vi "PicoScope5000aExampleRapidBlockBulkOverlapped.vi"() -> ()   [LabVIEW 2010]
uses:
  shared/PicoBuffers.ctl
  <vilib>/Waveform/DWDTOps.llb/DWDT Analog to Digital.vi
  PicoScope5000aLib/PicoScope5000aAnalogChannelSettings.ctl
  shared/Segment Range.ctl
  shared/Buffer and Transfer Settings.ctl
  shared/Acquisition Settings.ctl
  shared/nSegments.ctl
  PicoScope5000aLib/PicoScope5000aDigitalChannelSettings.ctl
panel:
  in  "Write TDMS file":bool
  out "Total Requested Samples":u64
  out "overflow":i16[](array[numeric]) format="%06b"
  in  "Port 0 Settings":T1={"Enabled"=FALSE, "Logic Level"=9830} {"Logic Level" items=["1.5V TTL"=9830, "2.5V CMOS"=16383]}
  in  "Channel A Settings":T2={"Enabled"=TRUE, "Coupling"=1, "Range"=6, "Analogue Offset"=0.0, "Bandwidth Limit"=0} {"Bandwidth Limit" items=["Full", "20MHz"]; "Range" items=["10 mV", "20 mV", "50 mV", "100 mV", "200 mV", "500 mV", "1 V", "2 V", "5 V", "10 V", "20 V"]; "Coupling" items=["AC", "DC"]}
  in  "Trigger Settings":T3={"Trigger Enabled"=FALSE, "Trigger Source"=enum."Channel A", "Trigger Threshold (volts)"=0.0, "Trigger Direction"=2, "Trigger Delay (samples)"=0, "Auto Trigger Time (ms)"=1000} {"Trigger Direction" items=["Rising"=2, "Falling"=3]}
  out "USB 3.0 device on non-USB 3.0 Port":bool=TRUE
  out "USB Powered":bool=TRUE
  out "Device Info":T4={"Driver Version"="0", "USB Version"="0", "Hardware"="0", "Variant"="0", "Batch and Serial"="0", "Cal Date"="0", "Kernel Version"="0", "Digital HW Version"="0", "Analogue HW Version"="0", "MSO"=FALSE, "Number of channels"=0}
  out "Trigger Offsets":cluster{"Samples":u64, "Time (seconds)":sgl}[](array[cluster]) {"Time (seconds)" format="%#_5p"}
  in  "Stop Display":bool
  out "Capture Complete":bool
  in  "Run":bool
  in  "Display Buffer Index":i32
  in  "Segment Range":T5={"fromSegmentIndex"=0, "toSegmentIndex"=9} {"toSegmentIndex" format="%.4p"; "fromSegmentIndex" format="%.4p"}
  in  "nSegments":T6=10 format="%.4p"
  out "error out":errorcluster
  in  "Data file":path=path "PicoScope5000aExampleRapidBlock"
  in  "Buffer and Transfer Settings":T7={"startIndex"=0, "Samples"=1000000, "Down Sample Ratio"=1, "Down-Sample Mode"=0} {"Down-Sample Mode" items=["None"=0, "Aggregate"=1, "Decimate"=2, "Average"=4, "RAW none"=2147483648]; "Down Sample Ratio" step=1; "Samples" format="%_6p"}
  in  "Acquisition Settings":T8={"preTriggerSamples"=0, "postTriggerSamples"=1000000, "timebase"=5} {"postTriggerSamples" format="%_6p"; "preTriggerSamples" format="%_6p"}
  out "Properties Panel":T9 {"Max Total Capture Time Available (sec)" format="%.3p"; "Sample Frequency" format="%.6p"; "Sample Rate" format="%.3p"; "Max Samples Available" format="%_6p"; "Total Capture Time (sec)" format="%.3p"}
  out "Port 0":digitalwaveform(graph)={"t0"=timestamp(0 s since 1904-01-01), "dt"=8e-09, "Y"={"transitions"=[], "data"=[]}}
  in  "stop":bool
  out "Analog Channels":cluster{i32, sgl, "Data":dbl[]}[](graph)
  in  "Resolution":u32(ring) items=["8-bit"=0, "12-bit"=1, "14-bit"=2, "15-bit"=3, "16-bit"=4, "10-bit"=10]
  in  "Serial Number":string
  in  "Use Serial Number":bool
  in  "error in (no error)":errorcluster
  # "Number of\nSegments to Capture"
  # "Bit 0 = ChA"
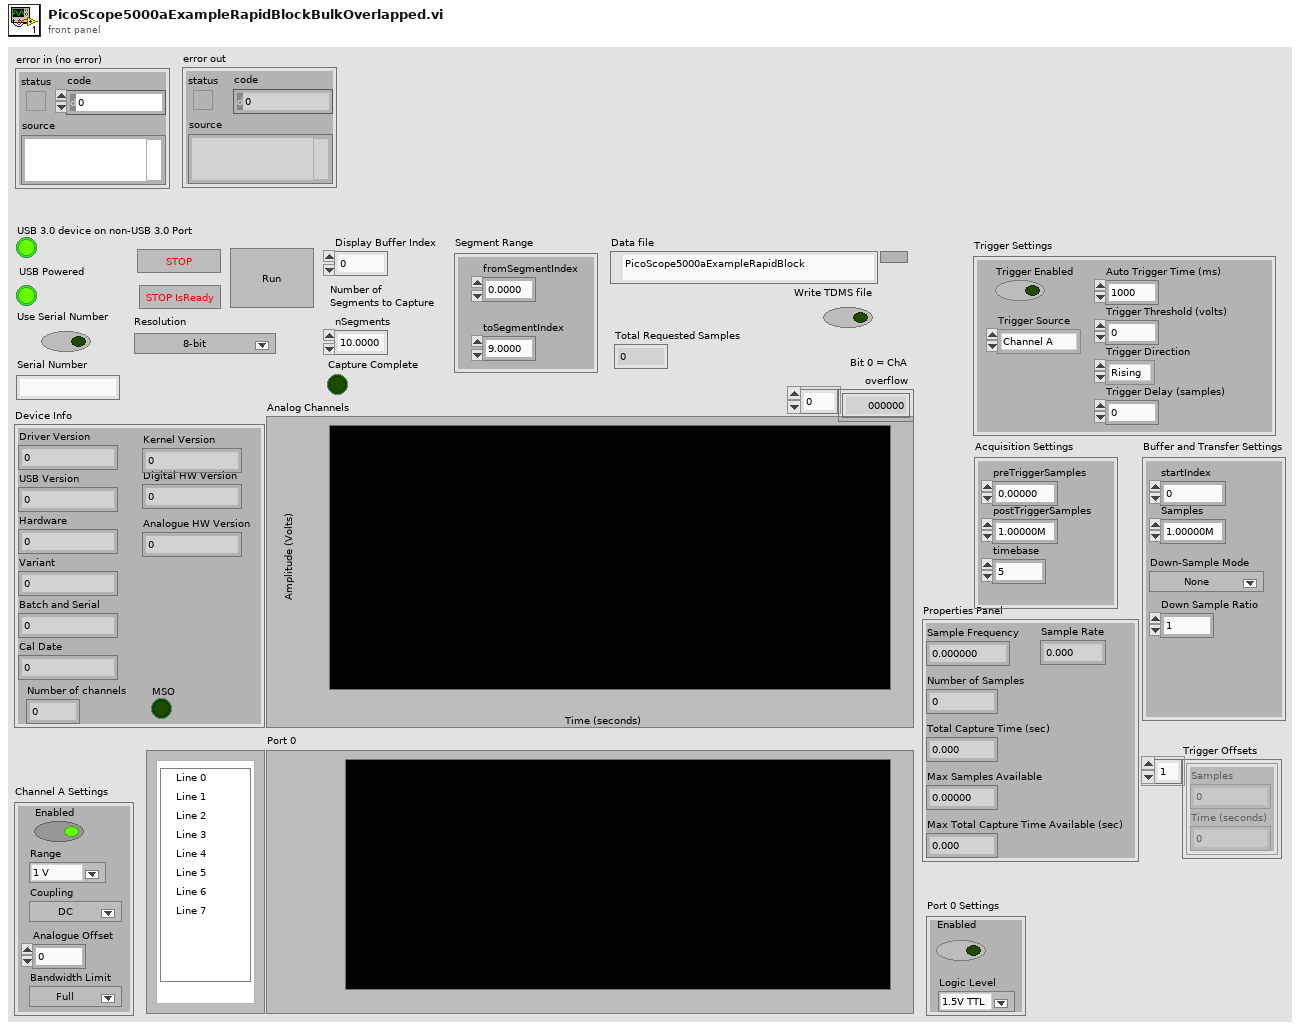
[diagram p1: front panel]
types:
  T1 = typedef "PicoScope5000aDigitalChannelSettings.ctl" = cluster{"Enabled":bool, "Logic Level":i16}
  T2 = typedef "PicoScope5000aAnalogChannelSettings.ctl" = cluster{"Enabled":bool, "Coupling":i16, "Range":u16, "Analogue Offset":sgl, "Bandwidth Limit":u32}
  T3 = cluster{"Trigger Enabled":bool, "Trigger Source":enum16{"Channel A", "Channel B", "Channel C", "Channel D", "Ext."}, "Trigger Threshold (volts)":dbl, "Trigger Direction":u16, "Trigger Delay (samples)":u32, "Auto Trigger Time (ms)":i16}
  T4 = cluster{"Driver Version":string, "USB Version":string, "Hardware":string, "Variant":string, "Batch and Serial":string, "Cal Date":string, "Kernel Version":string, "Digital HW Version":string, "Analogue HW Version":string, "MSO":bool, "Number of channels":i16}
  T5 = typedef "Segment Range.ctl" = cluster{"fromSegmentIndex":u64, "toSegmentIndex":u64}
  T6 = typedef "nSegments.ctl" = u64
  T7 = typedef "Buffer and Transfer Settings.ctl" = cluster{"startIndex":u64, "Samples":u64, "Down Sample Ratio":u64, "Down-Sample Mode":u32}
  T8 = typedef "Acquisition Settings.ctl" = cluster{"preTriggerSamples":u64, "postTriggerSamples":u64, "timebase":u32}
  T9 = cluster{"Sample Frequency":dbl, "Sample Rate":dbl, "Max Samples Available":u64, "Number of Samples":u64, "Total Capture Time (sec) ":dbl, "Max Total Capture Time Available (sec)":dbl}
  T10 = typedef "PicoBuffers.ctl" = cluster{"Max Buffer Pointers":u64[][][], "Min Buffer Pointers":u64[][][], "StreamingDataInfo":cluster{"Channel":u32, "Down-Sample Mode":u32, "PICO_DATA_TYPE":enum32{"PICO_INT8_T", "PICO_INT16_T", "PICO_INT32_T", "PICO_UINT32_T", "PICO_INT64_T", ""}, "Samples":i32, "bufferIndex":u64, "startIndex":i32, "overflow":i16}[][]}
  T11 = enum16{"open", "open or create", "create or replace", "create", "open (read-only)"}
  T12 = cluster{"Sample Frequency":sgl, "Sample Rate":sgl, "Max Samples Available":i32, "Number of Samples":u32, "Total Capture Time (sec) ":sgl, "Max Total Capture Time Available (sec)":sgl}
  T13 = cluster{"Channel A Buffer":i16[], "Channel B Buffer":i16[], "Channel C Buffer":i16[], "Channel D Buffer":i16[], "Channel E Buffer":i16[], "Channel F Buffer":i16[], "Channel G Buffer":i16[], "Channel H Buffer":i16[], "Port 0 Buffer":i16[], "Port 1 Buffer":i16[]}[]
  T14 = cluster{"Channel A Buffer":i16[], "Channel B Buffer":i16[], "Channel C Buffer":i16[], "Channel D Buffer":i16[], "Channel E Buffer":i16[], "Channel F Buffer":i16[], "Channel G Buffer":i16[], "Channel H Buffer":i16[], "Port 0 Buffer":i16[], "Port 1 Buffer":i16[]}
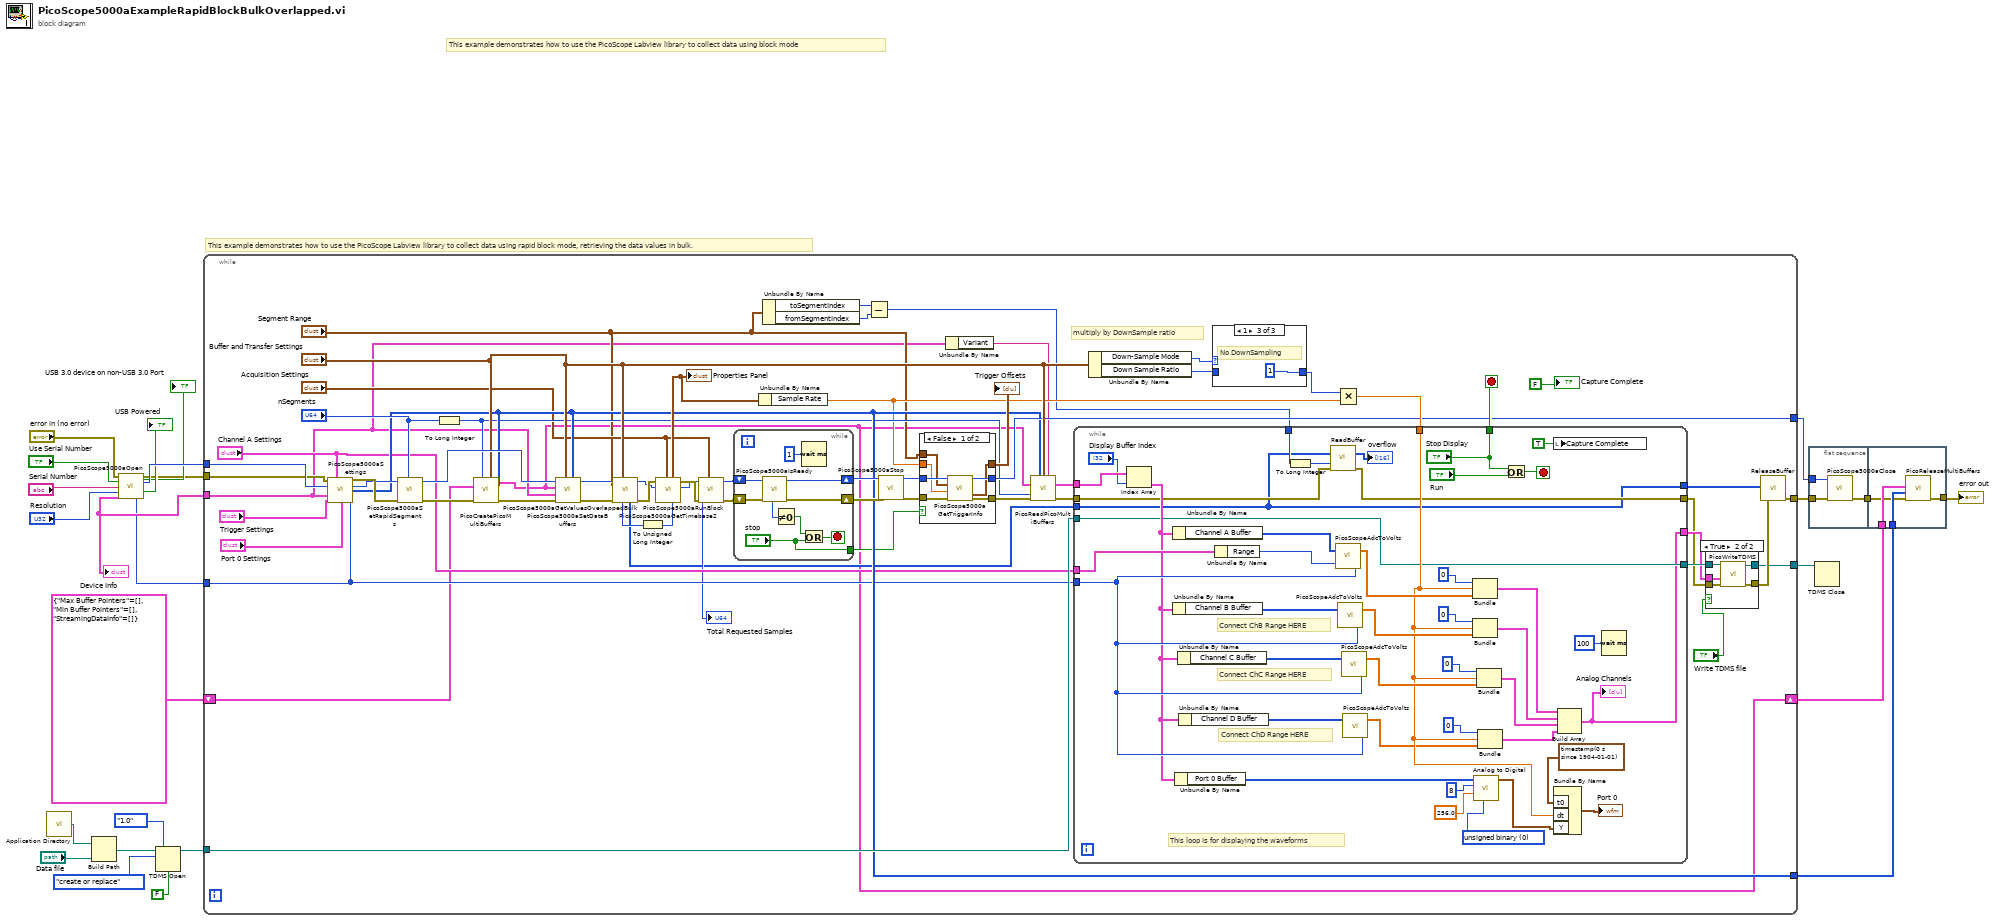
[diagram p0: block diagram]
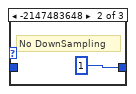
[diagram p5: hidden frame]
diagram:
  # "This example demonstrates how to use the PicoScope Labview library to collect data using rapid block mode, retrieving the data values in bulk."
  # "This example demonstrates how to use the PicoScope Labview library to collect data using block mode"
  n1 = call <vilib>:"Application Directory.vi"() -> ("Application Directory"=w19:path)
  n2 = Build Path(base path=w19, name or relative path="Data file") -> (appended path=w20:path)
  n3 = call "PicoScope5000aOpen.vi"("error in (no error)"="error in (no error)", "Serial Number"="Serial Number", "Use Serial Number"="Use Serial Number", "Resolution"="Resolution") -> ("USB 3.0 device on non-USB 3.0 Port"=→"USB 3.0 device on non-USB 3.0 Port":bool, "error out"=w8:errorcluster, "handle"=w25:i16, "USB Powered"=→"USB Powered":bool, "Device Info"=w12:T4, "Max ADC value"=w11:i16)  [unwired: 6 in]
  "Device Info" <- w12
  n4 = TDMS Open(6:FALSE ("disable buffering? (T)"), 7:enum16{"1.0", "2.0"}."1.0" ("file format version (2.0)"), 10:T11."create or replace" ("operation (0:open)"), 11:w20) -> (3:w17:refnum<k34>)  [unwired: 2 in, 1 out]
  n5 = while {
    tunnel: w25 -> [w56]
    tunnel: w11 -> [w48]
    tunnel: [w68] -> w6
    tunnel: [w53] -> w5
    tunnel: [w27] -> w18
    tunnel: w17 -> [w87]
    tunnel: w12 -> [w34]
    tunnel: w8 -> [w55]
    tunnel: [w41] -> w2
    shift-right: [w32] -> w4
    shift-left: T10 {"Max Buffer Pointers"=[], "Min Buffer Pointers"=[], "StreamingDataInfo"=[]} ("Data Pointers") -> [w33]
    stop <- w72 stop-if-true
    # "multiply by DownSample ratio"
    n6 = call "PicoScope5000aSettings.vi"("error in"=w55, "Channel A Settings"="Channel A Settings", "Port 0 Settings"="Port 0 Settings", "handle in"=w56, "Device Info"=w34, "Trigger Settings"="Trigger Settings", "Max ADC value"=w48) -> ("error out"=w58:errorcluster, "handle out"=w57:i16, "enabled array"=w53:i16[])  [unwired: 6 in]
    n7 = call "PicoScope5000aSetRapidSegments.vi"("nSegments"="nSegments", "error in (no error)"=w58, "handle in"=w57) -> ("error out"=w86:errorcluster, "handle out"=w85:i16)  [unwired: 6 in, 1 out]
    n8 = To Long Integer(number="nSegments") -> (32bit integer=w51:i32)
    n9 = call "PicoCreatePicoMultiBuffers.vi"("Number of Buffers"=w51, "Buffer and Transfer Settings"="Buffer and Transfer Settings", "enabled array"=w53, "Data Pointers In"=w33, "error in (no error)"=w86) -> ("Data Pointers"=w32:T10, "error out"=w88:errorcluster)  [unwired: 9 in]
    n10 = call "PicoScope5000aSetDataBuffers.vi"("enabled array"=w53, "Buffer and Transfer Settings"="Buffer and Transfer Settings", "error in (no error)"=w88, "Device Info"=w34, "Data Pointers In"=w32, "handle in"=w85) -> ("error out"=w84:errorcluster, "handle out"=w83:i16)  [unwired: 4 in]
    n11 = call "PicoScope5000aGetValuesOverlappedBulk.vi"("Segment Range"="Segment Range", "Buffer and Transfer Settings"="Buffer and Transfer Settings", "error in (no error)"=w84, "handle in"=w83) -> ("error out"=w62:errorcluster, "handle out"=w61:i16, "Pointer to Overflow"=w40:u64[], "noOfSamples"=w43:u64)  [unwired: 4 in]
    n12 = To Unsigned Long Integer(number=w43) -> (unsigned 32bit integer=w42:u32)
    n13 = call "PicoScope5000aGetTimebase2.vi"("Number of Samples"=w42, "Acquisition Settings"="Acquisition Settings", "handle in"=w61, "error in (no error)"=w62) -> ("handle out"=w59:i16, "error out"=w60:errorcluster, "Properties Panel"=w78:T12)  [unwired: 5 in]
    "Properties Panel" <- w78
    n14 = call "PicoScope5000aRunBlock.vi"("Acquisition Settings"="Acquisition Settings", "error in (no error)"=w60, "handle in"=w59) -> ("error out"=w75:errorcluster, "handle out"=w74:i16, "Total Requested Samples"=→"Total Requested Samples":u64)  [unwired: 5 in, 1 out]
    n15 = while {
      shift-right: [w155] -> w66
      shift-left: w75 -> [w156]
      shift-right: [w154] -> w63
      shift-left: w74 -> [w153]
      tunnel: ["stop"] -> w47
      stop <- w149 stop-if-true
      n16 = call "PicoScope5000aIsReady.vi"("error in (no error)"=w156, "handle in"=w153) -> ("error out"=w155:errorcluster, "handle out"=w154:i16, "ready"=w151:i16)  [unwired: 7 in]
      n17 = Not Equal To 0?(x=w151) -> (x != 0?=w150:bool)
      n18 = Wait (ms)(milliseconds to wait=u32 1) -> ()  [unwired: 1 out]
      n19 = Or(x=w150, y="stop") -> (x .or. y?=w149:bool)
    }
    n20 = Unbundle By Name(w78) -> ("Sample Rate"=w46:sgl)
    n21 = Unbundle By Name("Segment Range") -> ("toSegmentIndex"=w38:u64, "fromSegmentIndex"=w37:u64)
    n22 = Subtract(x=w38, y=w37) -> (x-y=w35:u64)
    n23 = call "PicoScope5000aStop.vi"("error in (no error)"=w66, "handle in"=w63) -> ("error out"=w65:errorcluster, "handle out"=w64:i16)  [unwired: 8 in]
    n24 = case shown="False" w47 {
      tunnel: [w102 w103] -> w69
      tunnel: [w101 w104] -> w68
      tunnel: [w100 _] -> w67
      tunnel: w65 -> [w99 w103]
      tunnel: w64 -> [w98 w104]
      tunnel: "Segment Range" -> [w97 _]
      tunnel: w46 -> [w96 _]
      frame False {
        n25 = call "PicoScope5000aGetTriggerInfo.vi"("handle in"=w98, "Rapid Block Acquisition Settings"=w97, "Sample Rate"=w96, "error in"=w99) -> ("handle out"=w101:i16, "Trigger Offsets"=w100:cluster{u64, sgl}[], "error out"=w102:errorcluster)  [unwired: 8 in, 1 out]
      }
      frame True {
      }
    }
    "Trigger Offsets" <- w67
    n26 = Unbundle By Name(w34) -> ("Variant"=w45:string)
    n27 = call "PicoReadPicoMultiBuffers.vi"("enabled array"=w53, "Buffer and Transfer Settings"="Buffer and Transfer Settings", "Variant"=w45, "Data Pointers"=w32, "No of Buffers"=w51, "error in (no error)"=w69) -> ("MultiBuffers (Max or non-aggregated)"=w81:T13, "error out"=w73:errorcluster)  [unwired: 7 in, 1 out]
    n28 = Unbundle By Name("Buffer and Transfer Settings") -> ("Down-Sample Mode"=w79:u32, "Down Sample Ratio"=w80:u64)
    n29 = case shown="1" w79 {
      tunnel: [w157 u64 1 ("Down Sample Ratio") u64 1 ("Down Sample Ratio")] -> w76
      tunnel: w80 -> [w157 _ _]
      frame Default {
      }
      frame -2147483648 {
        # "No DownSampling"
      }
      frame 1 {
        # "No DownSampling"
      }
    }
    n30 = Multiply(x=w76, y=w46) -> (x*y=w77:sgl)
    n31 = while {
      tunnel: w48 -> [w121]
      tunnel: "Channel A Settings" -> [w147]
      tunnel: w81 -> [w120]
      tunnel: w77 -> [w122]
      tunnel: [w111] -> w29
      tunnel: w73 -> [w112]
      tunnel: ["Stop Display"] -> w72
      tunnel: w40 -> [w108]
      tunnel: [w108] -> w39
      tunnel: w35 -> [w109]
      tunnel: w87 -> [w106]
      tunnel: [w106] -> w31
      tunnel: [w105] -> w30
      stop <- w130 stop-if-true
      w139 = u16 0 items=["unsigned binary", "offset binary", "2's complement"] ("data format (offset binary)")
      # "This loop is for displaying the waveforms"
      # "Connect ChB Range HERE"
      # "Connect ChD Range HERE"
      # "Connect ChC Range HERE"
      n32 = Index Array(array=w120, index="Display Buffer Index") -> (element=w114:T14)
      n33 = Unbundle By Name(w114) -> ("Channel A Buffer"=w115:i16[])
      n34 = Unbundle By Name(w114) -> ("Channel B Buffer"=w144:i16[])
      n35 = Unbundle By Name(w114) -> ("Port 0 Buffer"=w137:i16[])
      n36 = Unbundle By Name(w114) -> ("Channel C Buffer"=w126:i16[])
      n37 = Unbundle By Name(w114) -> ("Channel D Buffer"=w118:i16[])
      n38 = Unbundle By Name(w147) -> ("Range"=w116:u16)
      n39 = To Long Integer(number=w109) -> (32bit integer=w113:i32)
      n40 = call "ReadBuffer.vi"("Pointer and BufferSize"=w108, "Buffer size"=w113, "error in (no error)"=w112) -> ("Output Array"=→"overflow":i16[], "error out"=w111:errorcluster)  [unwired: 11 in]
      n41 = call "PicoScopeAdcToVolts.vi"("Max_adc"=w121, "Range Index"=w116, "Data"=w115) -> ("Data"=w133:dbl[])
      n42 = call "PicoScopeAdcToVolts.vi"("Max_adc"=w121, "Data"=w144) -> ("Data"=w143:dbl[])  [unwired: 1 in]
      n43 = call "PicoScopeAdcToVolts.vi"("Max_adc"=w121, "Data"=w126) -> ("Data"=w125:dbl[])  [unwired: 1 in]
      n44 = call "PicoScopeAdcToVolts.vi"("Max_adc"=w121, "Data"=w118) -> ("Data"=w117:dbl[])  [unwired: 1 in]
      n45 = Bundle(0, w122, "Data"=w133) -> (w142:cluster{i32, sgl, "Data":dbl[]})  [unwired: 1 in]
      n46 = Bundle(0, w122, "Data"=w143) -> (w141:cluster{i32, sgl, "Data":dbl[]})  [unwired: 1 in]
      n47 = call-poly <vilib>:"Analog to Digital.vi"("data format (offset binary)"=w139, "full-scale range (pk-pk)"=256.0, "resolution (16 bit)"=8, "analog waveform"=w137) -> ("digital waveform"=w134:digitalwaveform)  [unwired: 4 in, 3 out]
      n48 = Bundle(0, w122, "Data"=w125) -> (w124:cluster{i32, sgl, "Data":dbl[]})  [unwired: 1 in]
      n49 = Bundle(0, w122, "Data"=w117) -> (w107:cluster{i32, sgl, "Data":dbl[]})  [unwired: 1 in]
      n50 = Or(x="Stop Display", y="Run") -> (x .or. y?=w130:bool)
      n51 = local write "Capture Complete"(TRUE ("Capture Complete")) -> ()
      n52 = Bundle By Name("t0"=timestamp(0 s since 1904-01-01), "dt"=w122, "Y"=w134) -> (→"Port 0":digitalwaveform)  [unwired: 1 in]
      n53 = Build Array(w142, w141, w124, w107) -> (w105:cluster{i32, sgl, "Data":dbl[]}[])
      "Analog Channels" <- w105
      n54 = Wait (ms)(milliseconds to wait=u32 100) -> ()  [unwired: 1 out]
    }
    n55 = case shown="True" "Write TDMS file" {
      tunnel: w31 -> [w89 w95]
      tunnel: w30 -> [_ w94]
      tunnel: w29 -> [w90 w93]
      tunnel: [w90 w92] -> w28
      tunnel: [w89 w91] -> w27
      frame False {
      }
      frame True {
        n56 = call "PicoWriteTDMS.vi"("error in (no error)"=w93, "Analog Channels"=w94, "Refnum in"=w95) -> ("error out"=w92:errorcluster, "Refnum out"=w91:refnum<k34>)  [unwired: 7 in]
      }
    }
    n57 = call "ReleaseBuffer.vi"("error in (no error)"=w28, "Pointer and BufferSize"=w39) -> ("error out"=w41:errorcluster)  [unwired: 9 in]
    "Capture Complete" <- FALSE ("Capture Complete")
  }
  n58 = flat-sequence {
    tunnel: w6 -> [w162]
    tunnel: w2 -> [w161]
    tunnel: [w160] -> w1
    tunnel: w5 -> [w166]
    tunnel: w4 -> [w165]
    tunnel: [w164] -> w3
    tunnel: w1 -> [w163]
    frame #0 {
      n59 = call "PicoScope5000aClose.vi"("error in (no error)"=w161, "handle in"=w162) -> ("error out"=w160:errorcluster)  [unwired: 8 in, 1 out]
    }
    frame #1 {
      n60 = call "PicoReleaseMultiBuffers.vi"("error in (no error)"=w163, "Enabled array"=w166, "Data Pointers"=w165) -> ("error out"=w164:errorcluster)  [unwired: 7 in, 1 out]
    }
  }
  n61 = TDMS Close(11:w18) -> ()  [unwired: 1 in, 2 out]
  "error out" <- w3
